vi "GetPanelUI.vi"(8 "error in (no error)":errorcluster, 11 "object in":refnum<class "Template_CFG.lvclass">) -> (0 "error out":errorcluster, 2 "VI Refnum":refnum<vi>, 3 "object out":refnum<class "Template_CFG.lvclass">)   [LabVIEW 2021, in "Template-ChannelsChild.lvlib" / "Template_CFG.lvclass"]
uses:
  Template_CFG.lvclass
  Template_CFG.lvclass/Template_CFG.ctl
  TemplatePanel_Child.vi
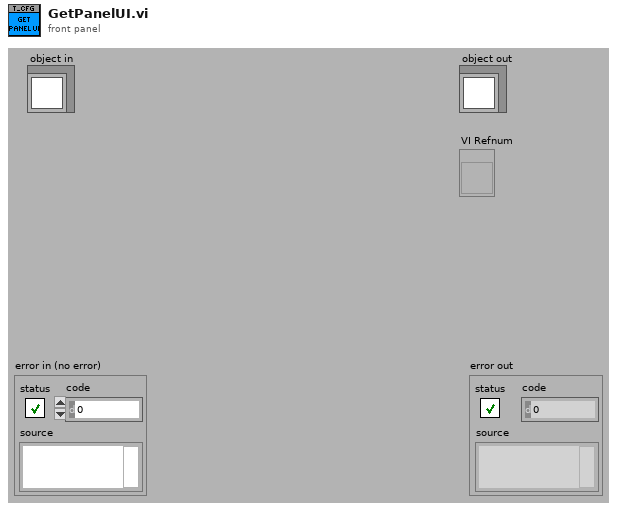
[diagram p1: front panel]
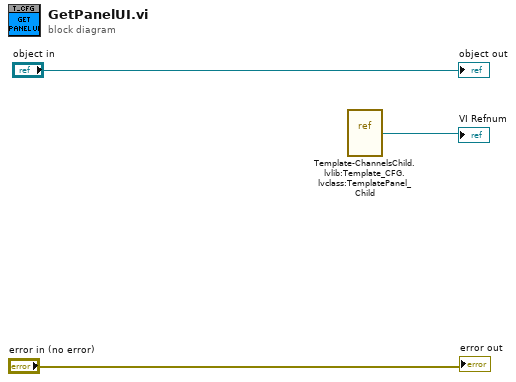
[diagram p0: block diagram]
diagram:
  n1 = vi-ref "Template-ChannelsChild.lvlib:Template_CFG.lvclass:TemplatePanel_Child.vi"() -> (→"VI Refnum":refnum<vi>)
  "error out" <- "error in (no error)"
  "object out" <- "object in"
